vi "Sous_VI_Virage_Gauche.vi"(8 "Angle rotation degres":i32, 11 "Choix rotation":T1) -> ()   [LabVIEW 2017]
uses:
  enum_rotation_robot.ctl
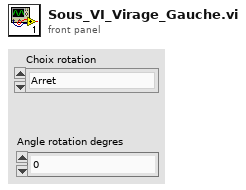
[diagram p1: front panel]
types:
  T1 = typedef "enum_rotation_robot.ctl" = enum16{"Arret", "Rotation_gauche", "Rotation_droite"}
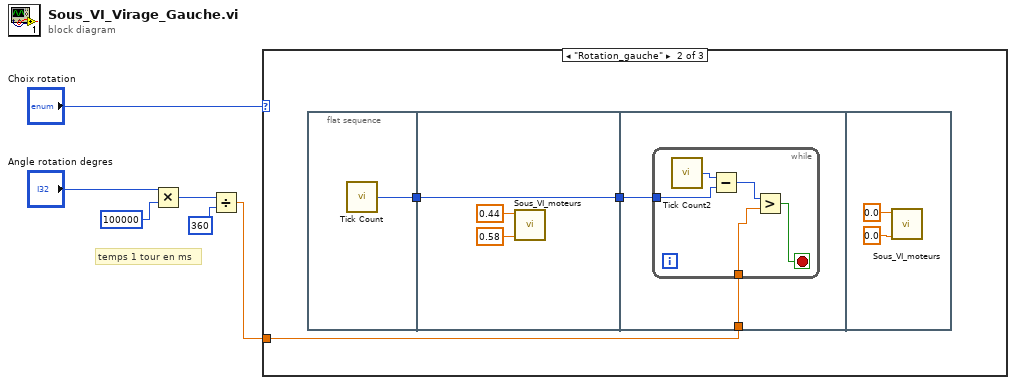
[diagram p0: block diagram]
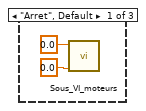
[diagram p2: hidden frame]
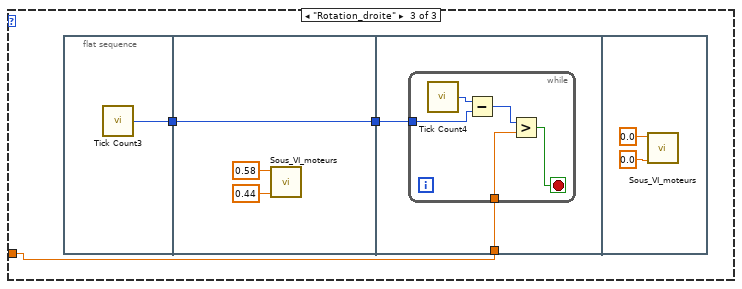
[diagram p3: hidden frame]
diagram:
  # "temps 1 tour en ms"
  n1 = Multiply(x="Angle rotation degres", y=100000) -> (x*y=w5:i32)
  n2 = Divide(x=w5, y=360) -> (x/y=w1:dbl)
  n3 = case shown="\"Rotation_gauche\"" "Choix rotation" {
    tunnel: w1 -> [_ w9 w25]
    frame "Arret", Default {
      n4 = call "Sous_VI_moteurs.vi"("Moteur Droit"=0.0, "Moteur Gauche"=0.0) -> ()  [unwired: 10 in]
    }
    frame "Rotation_gauche" {
      n5 = flat-sequence {
        tunnel: [w12] -> w10
        tunnel: [w13] -> w11
        tunnel: w10 -> [w13]
        tunnel: w11 -> [w17]
        tunnel: w9 -> [w16]
        frame #0 {
          n6 = call "Tick Count"() -> ("Tick Count(mSec)"=w12:u32)
        }
        frame #1 {
          n7 = call "Sous_VI_moteurs.vi"("Moteur Droit"=0.58, "Moteur Gauche"=0.44) -> ()  [unwired: 10 in]
        }
        frame #2 {
          n8 = while {
            tunnel: w17 -> [w21]
            tunnel: w16 -> [w19]
            stop <- w18 stop-if-true
            n9 = call "Tick Count2"() -> ("Tick Count(mSec)"=w22:u32)
            n10 = Subtract(x=w22, y=w21) -> (x-y=w20:u32)
            n11 = Greater?(x=w20, y=w19) -> (0:w18:bool)
          }
        }
        frame #3 {
          n12 = call "Sous_VI_moteurs.vi"("Moteur Droit"=0.0, "Moteur Gauche"=0.0) -> ()  [unwired: 10 in]
        }
      }
    }
    frame "Rotation_droite" {
      n13 = flat-sequence {
        tunnel: [w28] -> w27
        tunnel: [w31] -> w26
        tunnel: w27 -> [w31]
        tunnel: w26 -> [w33]
        tunnel: w25 -> [w32]
        frame #0 {
          n14 = call "Tick Count3"() -> ("Tick Count(mSec)"=w28:u32)
        }
        frame #1 {
          n15 = call "Sous_VI_moteurs.vi"("Moteur Droit"=0.44, "Moteur Gauche"=0.58) -> ()  [unwired: 10 in]
        }
        frame #2 {
          n16 = while {
            tunnel: w33 -> [w37]
            tunnel: w32 -> [w34]
            stop <- w35 stop-if-true
            n17 = call "Tick Count4"() -> ("Tick Count(mSec)"=w38:u32)
            n18 = Subtract(x=w38, y=w37) -> (x-y=w36:u32)
            n19 = Greater?(x=w36, y=w34) -> (0:w35:bool)
          }
        }
        frame #3 {
          n20 = call "Sous_VI_moteurs.vi"("Moteur Droit"=0.0, "Moteur Gauche"=0.0) -> ()  [unwired: 10 in]
        }
      }
    }
  }
